vi "Exec Every X ms.vi"(4 "Trigger interval (1000ms)":u32) -> (1 "Trigged?":bool)   [LabVIEW 2019]
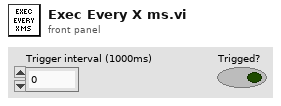
[diagram p1: front panel]
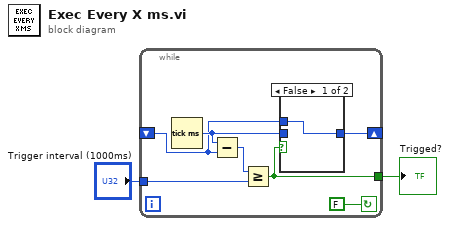
[diagram p0: block diagram]
diagram:
  n1 = while {
    shift-right: [w5] -> _
    shift-left: _ -> [w4]
    tunnel: "Trigger interval (1000ms)" -> [w8]
    tunnel: [w7] -> w2
    stop <- FALSE continue-if-true
    n2 = Tick Count (ms)() -> (millisecond timer value=w6:u32)
    n3 = Subtract(x=w6, y=w4) -> (x-y=w9:u32)
    n4 = Greater Or Equal?(x=w9, y=w8) -> (x >= y?=w7:bool)
    n5 = case shown="False" w7 {
      tunnel: w6 -> [_ w11]
      tunnel: [w10 w11] -> w5
      tunnel: w4 -> [w10 _]
      frame False {
      }
      frame True {
      }
    }
  }
  "Trigged?" <- w2
